vi "libssh2_sftp_fstatvfs.vi"(8 "error in (no error)":errorcluster, 11 "sftp handle":T2) -> (0 "error out":errorcluster, 2 "statvfs":T1)   [LabVIEW 2017, in "libssh2.lvlib"]
doc: "Get the file system information of a file handle."
uses:
  libssh2.lvlib
  SFTP Handle Refnum.ctl
  libssh2_sftp_statvfs.ctl
  Acquire SFTP.vi
  Release SFTP.vi
  Acquire Session.vi
  Release Session.vi
  Not An SFTP Handle Refnum.vi
  <vilib>/Utility/error.llb/Error Cluster From Error Code.vi
  Global Settings.vi
  Read SFTP Handle Refnum.vi
  Read SFTP Refnum.vi
  Read Session Refnum.vi
  <vilib>/Utility/semaphor.llb/Acquire Semaphore.vi
  <vilib>/Utility/semaphor.llb/Release Semaphore.vi
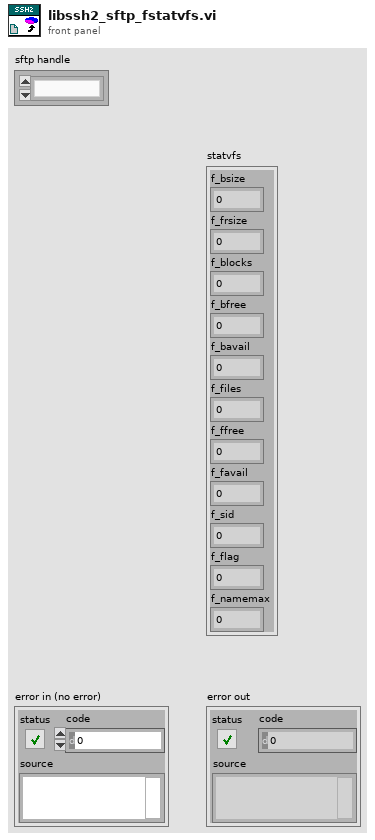
[diagram p1: front panel]
types:
  T1 = typedef "libssh2.lvlib/libssh2_sftp_statvfs.ctl" = cluster{"f_bsize":u64, "f_frsize":u64, "f_blocks":u64, "f_bfree":u64, "f_bavail":u64, "f_files":u64, "f_ffree":u64, "f_favail":u64, "f_sid":u64, "f_flag":u64, "f_namemax":u64}
  T2 = typedef "libssh2.lvlib/SFTP Handle Refnum.ctl" = refnum<k1>
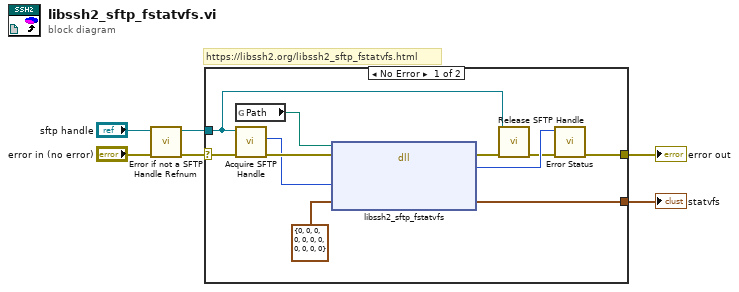
[diagram p0: block diagram]
diagram:
  # "https://libssh2.org/libssh2_sftp_fstatvfs.html"
  n1 = call "Error if not a SFTP Handle Refnum.vi"("error in (no error)"="error in (no error)", "sftp handle"="sftp handle") -> ("error out"=w5:errorcluster, "sftp handle out"=w4:T2)  [unwired: 8 in]
  n2 = case shown="No Error" w5 {
    selector: w5 -> [w16 w18]
    tunnel: w4 -> [w7 _]
    tunnel: [w12 w18] -> w3
    tunnel: [w9 _] -> w1
    frame No Error {
      n3 = global read "Global Settings.vi" "Path"() -> (w17:path)
      n4 = call "Acquire SFTP Handle.vi"("error in (no error)"=w16, "sftp handle"=w7) -> ("error out"=w15:errorcluster, "LIBSSH2_SFTP_HANDLE*"=w14:u64)  [unwired: 8 in]
      n5 = dll-call lib="?" fn="libssh2_sftp_fstatvfs"(path in=w17, error in=w15, "handle"=w14, "st"=T1 {"f_bsize"=0, "f_frsize"=0, "f_blocks"=0, "f_bfree"=0, "f_bavail"=0, "f_files"=0, "f_ffree"=0, "f_favail"=0, "f_sid"=0, "f_flag"=0, "f_namemax"=0} ("statvfs")) -> (error out=w13:errorcluster, "return value"=w11:i32, "st"=w9:T1)  [unwired: 2 in, 1 out]
      n6 = call "Release SFTP Handle.vi"("error in (no error)"=w13, "sftp handle"=w7) -> ("error out"=w8:errorcluster)  [unwired: 9 in]
      n7 = call "Error Status.vi"("error in (no error)"=w8, "return value"=w11) -> ("error out"=w12:errorcluster)  [unwired: 8 in, 1 out]
    }
    frame Error {
    }
  }
  "error out" <- w3
  "statvfs" <- w1
